vi "SEQU Gestion Fenetre Alerte.vi"(9 "Hauteur":i16, 11 "Largeur":i16) -> (1 "Left":i32, 3 "Top":i32)   [LabVIEW 2022 SP3]
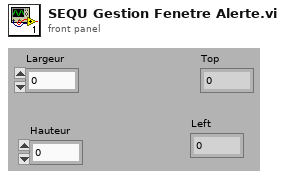
[diagram p1: front panel]
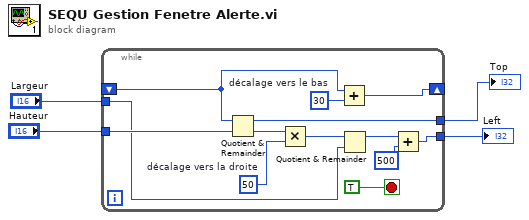
[diagram p0: block diagram]
diagram:
  n1 = while {
    shift-right: [w9] -> _
    shift-left: _ -> [w10]
    tunnel: "Hauteur" -> [w15]
    tunnel: "Largeur" -> [w11]
    tunnel: [w7] -> w2
    tunnel: [w8] -> w1
    stop <- TRUE stop-if-true
    w13 = 50  # décalage vers la droite
    w16 = 30  # décalage vers le bas
    n2 = Quotient & Remainder(x=w10, y=w15) -> (x-y*floor(x/y)=w8:i32, floor(x/y)=w14:i32)
    n3 = Multiply(x=w14, y=w13) -> (x*y=w12:i32)
    n4 = Add(x=w10, y=w16) -> (x+y=w9:i32)
    n5 = Quotient & Remainder(x=w12, y=w11) -> (x-y*floor(x/y)=w6:i32)  [unwired: 1 out]
    n6 = Add(x=w6, y=500) -> (x+y=w7:i32)
  }
  "Left" <- w2
  "Top" <- w1
